vi "3_VisualAD_Report(Dataset).vi"(0 "NNPC_Paths":T10={"CFG"=path "D:/Ngene/GitHub/deepltk_examples/3_Image_Processing/36_Anomaly_Detection/Models/3OfSpades/NNPC_3OfSpades.cfg", "BIN"=path "D:/Ngene/GitHub/deepltk_examples/3_Image_Processing/36_Anomaly_Detection/Models/3OfSpades/NNPC_3OfSpades.bin"}, 1 "NNPC_Setup":T1={"Input_Dims"={"C"=-1, "H"=-1, "W"=-1}, "mBatch"=1, "Device"=enum."GPU", "GPU Id"=0}, 2 "Feature_Scorer_Params":T12={"Nearest_Neighbors"=1, "Calculate Anomaly Map"=TRUE, "Gaussian_Blur"={"Kernel_Size"=33, "Sigma"=4.0}}, 5 "Dest. Path":path=path "D:/working/Results", 12 "Image_Dataset_Folder_Path":path=path "D:/Ngene/GitHub/deepltk_examples/3_Image_Processing/36_Anomaly_Detection/Dataset/Cards_3OfSpades/test", 13 "Ground_Truth_Folder_Path":path) -> ()   [LabVIEW 2020]
uses:
  <vilib>/Ngene/DeepLTK Anomaly Detection Addon/Toolkit/API/Controls/Feature_Scorer_Params.ctl
  <vilib>/Ngene/DeepLTK Anomaly Detection Addon/Toolkit/API/Controls/Gaussian_Blur.ctl
  <vilib>/Ngene/DeepLTK Anomaly Detection Addon/Toolkit/API/Controls/NN_Paths.ctl
  subVIs/Visualizer/Controls/Display_Options.ctl
  subVIs/Visualizer/Controls/ROI_Display_Options.ctl
  subVIs/Visualizer/Controls/Heatmap_Display_Options.ctl
  subVIs/Visualizer/Controls/ColorMap.ctl
  <vilib>/Ngene/DeepLTK Anomaly Detection Addon/Toolkit/API/Controls/MinMax.ctl
  subVIs/Visualizer/Controls/Report_Images_CFG.ctl
  <vilib>/Ngene/DeepLTK Anomaly Detection Addon/Toolkit/API/Controls/NNPC_Setup.ctl
  <vilib>/Ngene/Deep Learning Toolkit/Toolkit/NN_Data/API/NN_Dims(C,H,W).ctl
  <vilib>/Ngene/Deep Learning Toolkit/Toolkit/NN_Network/Controls/NN_Device.ctl
  <vilib>/Analysis/baseanly.llb/Mean (DBL).vi
  <vilib>/Ngene/DeepLTK Anomaly Detection Addon/Toolkit/API/NNPC_Predict/NNPC_Predict(Single).vi
  <vilib>/Ngene/DeepLTK Anomaly Detection Addon/Toolkit/DeepLTK_Anomaly_Detection_Addon.lvlib
  <vilib>/Analysis/NI_AALBase.lvlib
  <vilib>/Ngene/Deep Learning Toolkit/Toolkit/Deep_Learning_Toolkit_by_Ngene.lvlib
panel:
  in  "Display_Options":T4={"ROI_Options"={"Color"=16717824, "Width"=3, "Drawing Mode"=enum."Frame"}, "Heatmap_Options"={"ColorMap"=enum."Jet", "Alpha"=0.4, "Heatmap Range"={"Min"=17.0, "Max"=19.0}}, "Report_Images_CFG"={"Original Image"=TRUE, "Ground Truth"=FALSE, "HeatMap"=TRUE, "Mask"=TRUE, "Segmentation"=TRUE}} {"Heatmap_Options"."Heatmap Range"."Min" format="%#_5g"}
  out "Detection Results":T11(plugin-control)
  out "dt_Predict":dbl=0.013626885416698542 format="%#_4p"
  out "Actual_Pixel_Threshold":sgl=18.1
  out "Total":i32=48
  out "Progress":i32=47
  out "dT_ImRead":dbl=0.008457522916671678 format="%#_4p"
  in  "Pixel_Thrshld(Custom)":sgl=18.1 format="%_5g"
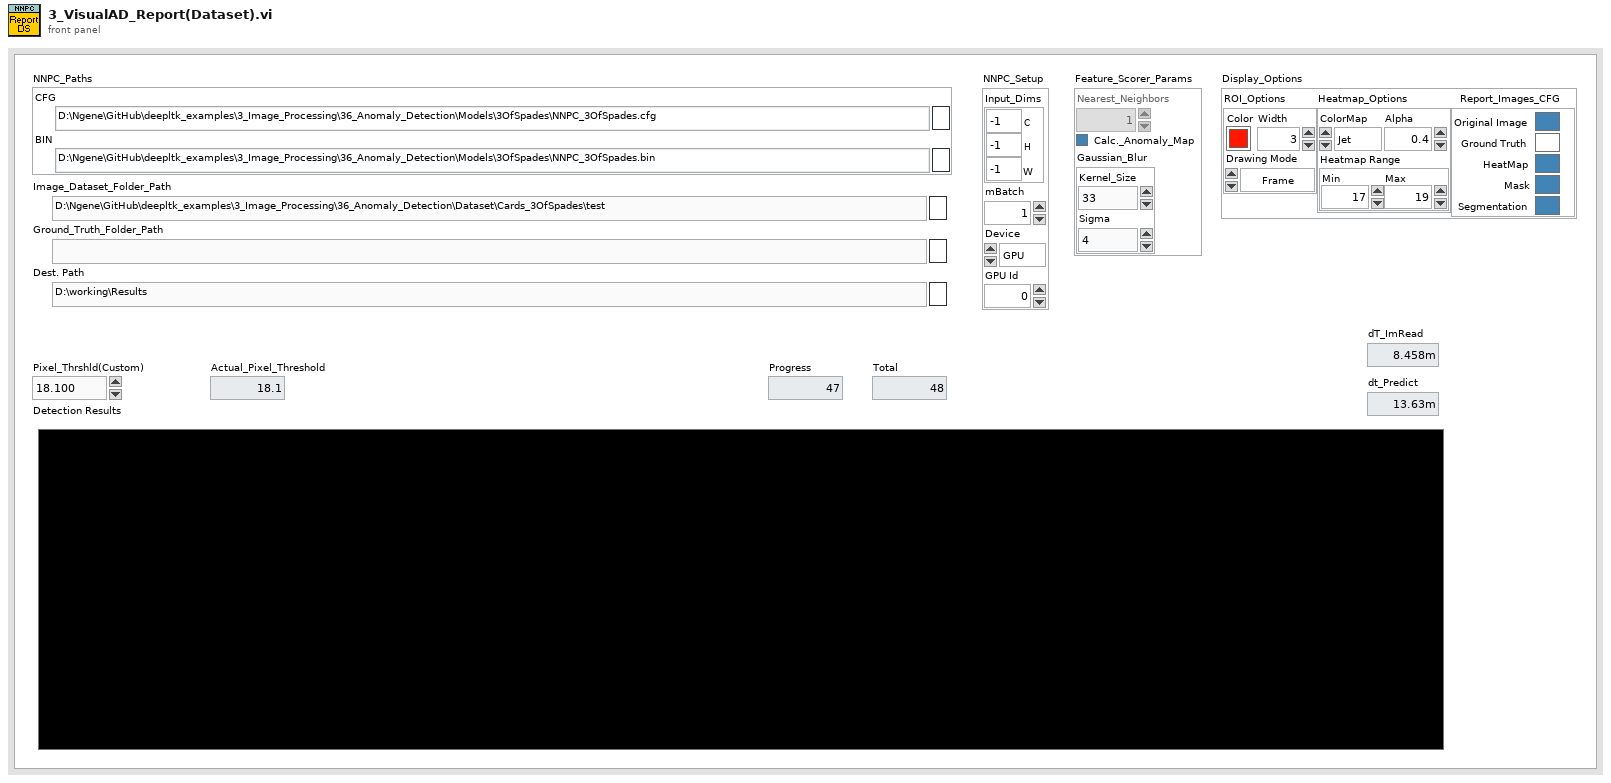
[diagram p1: front panel]
types:
  T1 = typedef "DeepLTK_Anomaly_Detection_Addon.lvlib/NNPC_Setup.ctl" = cluster{"Input_Dims":T2, "mBatch":i32, "Device":T3, "GPU Id":i32}
  T2 = typedef "Deep_Learning_Toolkit_by_Ngene.lvlib/NN_Dims(C,H,W).ctl" = cluster{"C":i32, "H":i32, "W":i32}
  T3 = typedef "Deep_Learning_Toolkit_by_Ngene.lvlib/NN_Device.ctl" = enum16{"CPU", "GPU"}
  T4 = typedef "Display_Options.ctl" = cluster{"ROI_Options":T5, "Heatmap_Options":T6, "Report_Images_CFG":T9}
  T5 = typedef "ROI_Display_Options.ctl" = cluster{"Color":u32, "Width":u32, "Drawing Mode":enum16{"Frame", "Fill"}}
  T6 = typedef "Heatmap_Display_Options.ctl" = cluster{"ColorMap":T7, "Alpha":sgl, "Heatmap Range":T8}
  T7 = typedef "ColorMap.ctl" = enum16{"Jet", "Perula", "Inferno", "Plasma", "Viridis"}
  T8 = typedef "DeepLTK_Anomaly_Detection_Addon.lvlib/MinMax.ctl" = cluster{"Min":sgl, "Max":sgl}
  T9 = typedef "Report_Images_CFG.ctl" = cluster{"Original Image":bool, "Ground Truth":bool, "HeatMap":bool, "Mask":bool, "Segmentation":bool}
  T10 = typedef "DeepLTK_Anomaly_Detection_Addon.lvlib/NN_Paths.ctl" = cluster{"CFG":path, "BIN":path}
  T11 = typedef "IMAQ Image.ctl" = refnum<image>
  T12 = typedef "DeepLTK_Anomaly_Detection_Addon.lvlib/Feature_Scorer_Params.ctl" = cluster{"Nearest_Neighbors":i32, "Calculate Anomaly Map":bool, "Gaussian_Blur":T13}
  T13 = typedef "DeepLTK_Anomaly_Detection_Addon.lvlib/Gaussian_Blur.ctl" = cluster{"Kernel_Size":i32, "Sigma":sgl}
  T14 = typedef "DeepLTK_Anomaly_Detection_Addon.lvlib/NNPC_Evaluation_Results.ctl" = cluster{"Threshold(Image)":sgl, "Threshold(Pixel)":sgl, "Pixel_Range":cluster{"Min":sgl, "Max":sgl}}
  T15 = typedef "DeepLTK_Anomaly_Detection_Addon.lvlib/NNPC_PreProcessing_Options.ctl" = cluster{"DS_Name":string, "Input_Dims":T2, "Cropping":T16, "Interpolation Type":u32, "MultiStage_ReSample?":bool, "Dataset_Stats":T17}
  T16 = typedef "DeepLTK_Anomaly_Detection_Addon.lvlib/Crop_CFG.ctl" = cluster{"Left":sgl, "Top":sgl, "Right":sgl, "Bottom":sgl}
  T17 = typedef "DeepLTK_Anomaly_Detection_Addon.lvlib/NNPC_DS_Stats.ctl" = cluster{"means":T18, "stds":T18}
  T18 = typedef "DeepLTK_Anomaly_Detection_Addon.lvlib/Image_Stats_RGB.ctl" = cluster{"R":sgl, "G":sgl, "B":sgl}
  T19 = typedef "DeepLTK_Anomaly_Detection_Addon.lvlib/NNPC_Instance.ctl" = cluster{"Name":string, "NN":T20, "MemBank_Data":T34}
  T20 = typedef "Deep_Learning_Toolkit_by_Ngene.lvlib/NN.ctl" = cluster{"Name":string, "No of Layers":i32, "mBatch":i32, "Layers":T21[], "Dimty":T22, "Dims_In":T2, "Dims_Out":T2, "Working_Dir":path, "Train?":bool, "Train_Params":T23, "LR_Update_Policy":T26, "Session Data":T28, "Ground_truth":T29, "NNg_hdls":T30, "NN_Device":T3, "GPU Id":i32, "Labels":string[], "Loss_Type":T31, "Loss_Cfg_Prms":variant, "NNG_WS":T32, "DryRun?":bool}
  T21 = typedef "Deep_Learning_Toolkit_by_Ngene.lvlib/NN_Layer_ref.ctl" = refnum<file>
  T22 = typedef "Deep_Learning_Toolkit_by_Ngene.lvlib/NN_In_Out_Dim-ty.ctl" = enum8{"In1D_Out1D", "In3D_Out1D", "In3D_Out3D", "In3D_OutBBox"}
  T23 = typedef "Deep_Learning_Toolkit_by_Ngene.lvlib/NN_Train_Params.ctl" = cluster{"Optimizer":T24, "Beta_1":sgl, "Beta_2":sgl, "Weight Decay(L1)":sgl, "Weight Decay(L2)":sgl, "Data_Sampling":T25}
  T24 = typedef "Deep_Learning_Toolkit_by_Ngene.lvlib/NN_Train_Optimizer.ctl" = enum16{"SGD", "Adam", "Adagrad", "Adadelta", "RMSProp", "Nesterov"}
  T25 = typedef "Deep_Learning_Toolkit_by_Ngene.lvlib/NN_Train_Data_Sampling.ctl" = enum16{"Random", "Sequential"}
  T26 = typedef "Deep_Learning_Toolkit_by_Ngene.lvlib/NN_LR_Policy_Cfg.ctl" = cluster{"Policy_Type":T27, "LR0":dbl, "k":sgl, "WarmUp_Policy":enum16{"Step", "Ramp"}, "WarmUp_Iter":i32, "WarmUp_Ratio":sgl}
  T27 = typedef "Deep_Learning_Toolkit_by_Ngene.lvlib/NN_LR_Policy_Type.ctl" = enum16{"Manual", "Step", "Exp", "1/t"}
  T28 = typedef "Deep_Learning_Toolkit_by_Ngene.lvlib/NN_Train_Session_Data.ctl" = cluster{"Epochs":sgl, "Tot_Iter":i32, "LR":sgl, "LR_iter":i32}
  T29 = typedef "Deep_Learning_Toolkit_by_Ngene.lvlib/NN_Ground_truth.ctl" = cluster{"Y":variant}
  T30 = typedef "Deep_Learning_Toolkit_by_Ngene.lvlib/nng_cuda_handles.ctl" = cluster{"cudnn":u64, "cublas":u64, "stream":u64, "curand":u64}
  T31 = typedef "Deep_Learning_Toolkit_by_Ngene.lvlib/NN_Loss_Type.ctl" = enum16{"None", "MSE", "CrossEntropy", "YOLO_v2", "YOLO_v4"}
  T32 = typedef "Deep_Learning_Toolkit_by_Ngene.lvlib/NNG_WS.ctl" = cluster{"NNG_WS_Mem":T33, "Max_WS_Size":i64}
  T33 = typedef "Deep_Learning_Toolkit_by_Ngene.lvlib/NNg_WS_Mem_DVR.ctl" = refnum<data-value>
  T34 = typedef "DeepLTK_Anomaly_Detection_Addon.lvlib/MemBank_and_Norm_Variants.ctl" = cluster{"MemBank":variant, "MemBank Norm":variant}
  T35 = typedef "Anomaly_Detection_Results_Imgs.ctl" = cluster{"Image":T11, "Ground Truth":T11, "Predicted Heat Map":T11, "Predicted Mask":T11, "Segmentation":T11}
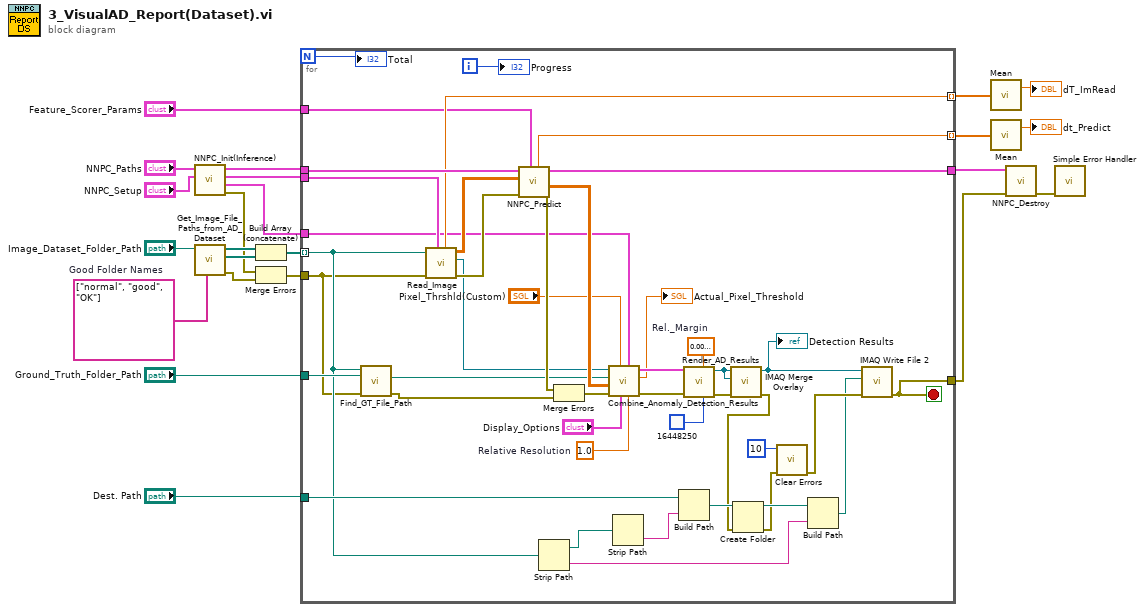
[diagram p0: block diagram]
diagram:
  w1 = string[] ["normal", "good", "OK"]  # Good Folder Names
  n1 = call <vilib>:"NNPC_Init(Inference).vi"("NNPC_Setup"="NNPC_Setup", "NNPC_Paths"="NNPC_Paths") -> ("error out"=w7:errorcluster, "Evaluation_Results"=w3:T14, "PreProc_Options"=w5:T15, "NNPC_out"=w20:T19)  [unwired: 5 in, 1 out]
  n2 = call "Get_Image_File_Paths_from_AD_Dataset.vi"("Good Folder Names"=w1, "Dataset Folder"="Image_Dataset_Folder_Path") -> ("error out"=w19:errorcluster, "Bad Dataset Files"=w13:path[], "Good Dataset Files"=w14:path[])  [unwired: 7 in]
  n3 = Build Array (concatenate)(w14, w13) -> (w12:path[])
  n4 = Merge Errors(w7, w19) -> (w6:errorcluster)
  n5 = for {
    N -> [w49]
    tunnel: w12 -> [w44] mode=indexing
    tunnel: w20 -> [w61]
    tunnel: [w64] -> w9
    tunnel: [w58] -> w17 mode=indexing
    tunnel: [w45] -> w16 mode=indexing
    tunnel: "Dest. Path" -> [w56]
    tunnel: "Ground_Truth_Folder_Path" -> [w47]
    tunnel: "Feature_Scorer_Params" -> [w41]
    tunnel: w5 -> [w35]
    tunnel: w3 -> [w34]
    tunnel: w6 -> [w38]
    tunnel: [w55] -> w22
    i -> [w50]
    stop <- w55 stop-if-true
    w24 = sgl 1.0  # Relative Resolution
    w32 = sgl 0.01  # Rel._Margin
    n6 = call "Find_GT_File_Path.vi"("error in"=w38, "GT Mask Folder Path"=w47, "Image File Path"=w44) -> ("error out"=w36:errorcluster, "GT File Path"=w46:path)  [unwired: 5 in, 2 out]
    n7 = call "Read_Image.vi"("PreProcessing_Options"=w35, "error in"=w38, "Img Path"=w44) -> ("error out"=w60:errorcluster, 2:"Image Out (Preproc)"=w31:T11, 3:"Image Out (Preproc)"=w40:sgl[][][], "dT_Img_Read"=w58:dbl)  [unwired: 3 in, 2 out]
    n8 = call-poly <vilib>:"NNPC_Predict.vi"("Feature_Scorer_Params"=w41, "error in"=w60, "Image_in"=w40, "NNPC_in"=w61) -> ("error out"=w65:errorcluster, "Anomaly_Map"=w63:sgl[][], "NNPC_out"=w64:T19, "dT_Predict"=w45:dbl)  [unwired: 2 in, 2 out]
    n9 = Strip Path(path=w44) -> (stripped path=w57:path, name=w33:string)
    n10 = Merge Errors(w65, w36) -> (w37:errorcluster)
    n11 = call "Combine_Anomaly_Detection_Results.vi"("Relative Resolution"=w24, "Evaluation_Results"=w34, "Display_Options"="Display_Options", "Pixel Anomaly Thrshld"="Pixel_Thrshld(Custom)", "error in"=w37, "Anomaly Map"=w63, "Gt File Path"=w46, "Orig Image In"=w31) -> ("error out"=w39:errorcluster, "Actual Pixel Threshold"=→"Actual_Pixel_Threshold":sgl, "Anomaly Detection Results"=w62:T35)  [unwired: 1 in]
    n12 = Strip Path(path=w57) -> (name=w42:string)  [unwired: 1 out]
    n13 = Build Path(base path=w56, name or relative path=w42) -> (appended path=w43:path)
    n14 = call "Render_AD_Results.vi"("Background Color"=u32 16448250, "Rel._Margin"=w32, "error in"=w39, "Anomaly Detection Rresults"=w62) -> ("error out"=w28:errorcluster, "Anomaly Detection Result"=w29:T11)  [unwired: 6 in]
    n15 = call "IMAQ Merge Overlay"("error in (no error)"=w28, "Image Dst"=w29, "Image Src"=w29) -> ("error out"=w27:errorcluster, "Image Dst Out"=w26:T11)  [unwired: 7 in]
    "Detection Results" <- w26
    n16 = Create Folder(path (use dialog)=w43, error in=w27) -> (created path=w53:path, error out=w52:errorcluster)  [unwired: 1 in, 1 out]
    n17 = call <vilib>:"Clear Errors.vi"("error in (no error)"=w52, "specific error code to clear (0: all)"=10) -> ("error out"=w66:errorcluster)  [unwired: 4 in, 1 out]
    n18 = Build Path(base path=w53, name or relative path=w33) -> (appended path=w54:path)
    n19 = call-poly "IMAQ Write File 2"("error in (no error)"=w66, "File Path"=w54, "Image"=w26) -> ("error out"=w55:errorcluster)  [unwired: 7 in, 1 out]
    "Progress" <- w50
    "Total" <- w49
  }
  n20 = call-poly <vilib>:"Mean.vi"("X"=w17) -> ("mean"=→"dT_ImRead":dbl)  [unwired: 1 out]
  n21 = call-poly <vilib>:"Mean.vi"("X"=w16) -> ("mean"=→"dt_Predict":dbl)  [unwired: 1 out]
  n22 = call <vilib>:"NNPC_Destroy.vi"("error in"=w22, "NNPC_in"=w9) -> ("error out"=w21:errorcluster)  [unwired: 9 in]
  n23 = call <vilib>:"Simple Error Handler.vi"("error in (no error)"=w21) -> ()  [unwired: 4 in, 5 out]
